vi "Single Tone Audio Measurements.vi"(6 "units settings":T1, 8 "error in":errorcluster, 10 "measurement settings":T4={"Band start"=20.0, "Band stop"=20000.0, "Amplitude"=1.0, "Frequency"=1000.0, "Full scale range"=3.16}, 11 "waveform":waveform(dbl)) -> (0 "error out":errorcluster, 1 "spectrum":cluster{"x0":dbl, "dx":dbl, "magnitude":dbl[]}, 2 "time domain":waveform(dbl), 3 "results":T5)   [LabVIEW 2021]
uses:
  <vilib>/addons/Sound and Vibration/svt_Single Tone Measurements/SoundVib_SingleTone.lvlib
  <vilib>/addons/Sound and Vibration/svt_Distortion/SoundVib_Distortion.lvlib
  controls/single tone audio measurements.ctl
  controls/audio controls.lvlib
  controls/units - ratio.ctl
  <vilib>/addons/Sound and Vibration/svt_Distortion/SVT SNR without Harmonics (Frequency) (1 Ch).vi
  <vilib>/addons/Sound and Vibration/svt_Single Tone Measurements/SVT Dynamic Range (Frequency) (1 Ch).vi
  <vilib>/addons/_NISVFA/_Shared subVIs/Common/SVL Set dB Reference (1 Ch).vi
  <vilib>/addons/Sound and Vibration/svt_Single Tone Measurements/SVT Gain (Time) (1 Ch).vi
  <vilib>/addons/_NISVFA/_Spectrum Processing/SVFA Unit Conversion (Complex) (1 Ch).vi
  <vilib>/addons/Sound and Vibration/svt_Single Tone Measurements/SVT Spurious Free Dynamic Range (Frequency) (1 Ch).vi
  controls/units - snr.ctl
  controls/units settings.ctl
  controls/single tone audio measurement settings.ctl
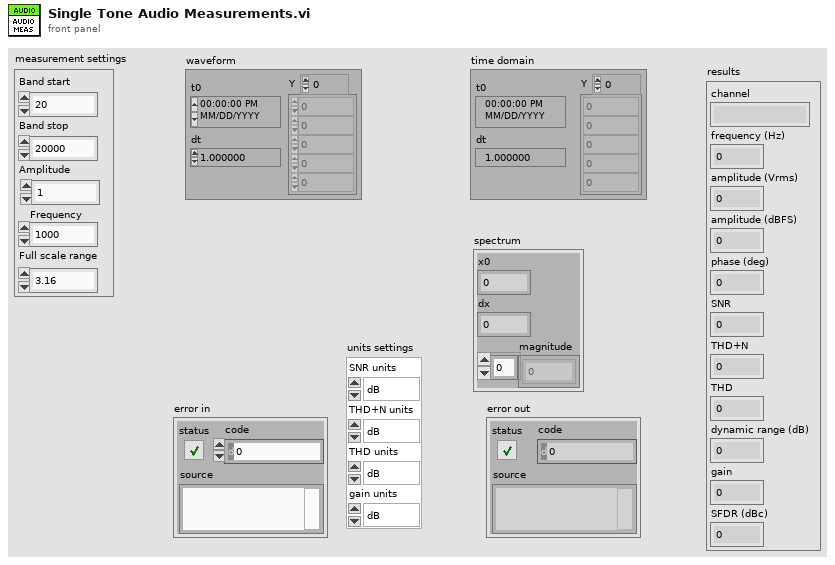
[diagram p1: front panel]
types:
  T1 = typedef "audio controls.lvlib/units settings.ctl" = cluster{"SNR units":T2, "THD+N units":T3, "THD units":T3, "gain units":T3}
  T2 = typedef "audio controls.lvlib/units - snr.ctl" = enum32{"dB", "x/y"}
  T3 = typedef "audio controls.lvlib/units - ratio.ctl" = enum32{"dB", "%", "x/y"}
  T4 = typedef "single tone audio measurement settings.ctl" = cluster{"Band start":dbl, "Band stop":dbl, "Amplitude":dbl, "Frequency":dbl, "Full scale range":dbl}
  T5 = typedef "audio controls.lvlib/single tone audio measurements.ctl" = cluster{"channel":string, "frequency (Hz)":dbl, "amplitude (Vrms)":dbl, "amplitude (dBFS)":dbl, "phase (deg)":dbl, "SNR":dbl, "THD+N":dbl, "THD":dbl, "dynamic range (dB)":dbl, "gain":dbl, "SFDR (dBc)":dbl}
  T6 = enum16{"no change", "spectrum", "spectral density"}
  T7 = cluster{"linear/dB":enum16{"no change", "linear", "dB"}, "dB reference (0: no change)":dbl, "power/magnitude":enum16{"no change", "power", "magnitude"}, "view":enum16{"no change", "rms", "peak", "peak-peak"}}
  T8 = cluster{"start frequency":dbl, "stop frequency":dbl}
  T9 = cluster{"gain units":enum16{"dB", "linear ratio"}, "detected fundamental amplitude units":enum16{"EU rms", "EU peak", "EU peak-peak"}}
  T10 = cluster{"SNR units":enum16{"dB", "linear ratio", "%"}, "detected fundamental amplitude units":enum16{"EU rms", "EU peak", "EU peak-peak"}}
  T11 = typedef "svc_Spectrum Info.ctl" = cluster{"channel name":string, "description":string, "x-axis units":T12, "spectral info":cluster{"spectrum type":T13, "linear/dB":enum16{"linear", "dB"}, "window":u16, "window size":i32, "FFT size":i32}, "engineering units":T14, "custom label":string, "dB reference [EU]":dbl, "peak units":enum16{"rms", "peak", "peak-peak"}, "weighting filter":T15, "spectral density?":bool, "unit label":string, "spectrum skewed?":bool, "complimentary spectrum units":T16}
  T12 = typedef "svc_X-Axis Units.ctl" = u16
  T13 = typedef "svc_Spectrum Type.ctl" = enum16{"FFT Spectrum [complex]", "Amplitude [Magnitude]", "Power [Magnitude^2]", "Cross Spectrum [complex]", "Frequency Response [Complex]"}
  T14 = typedef "svc_Engineering Units Text Ring.ctl" = u16
  T15 = typedef "svc_Weighting Filter Text Ring.ctl" = u16
  T16 = typedef "svc_Complimentary Spectrum Units.ctl" = enum16{"none", "radians", "degrees", "cycles", "imaginary"}
  T17 = cluster{"complex spectrum response":cluster{"f0":dbl, "df":dbl, "complex spectrum":cdb[]}, "spectrum info":T11}
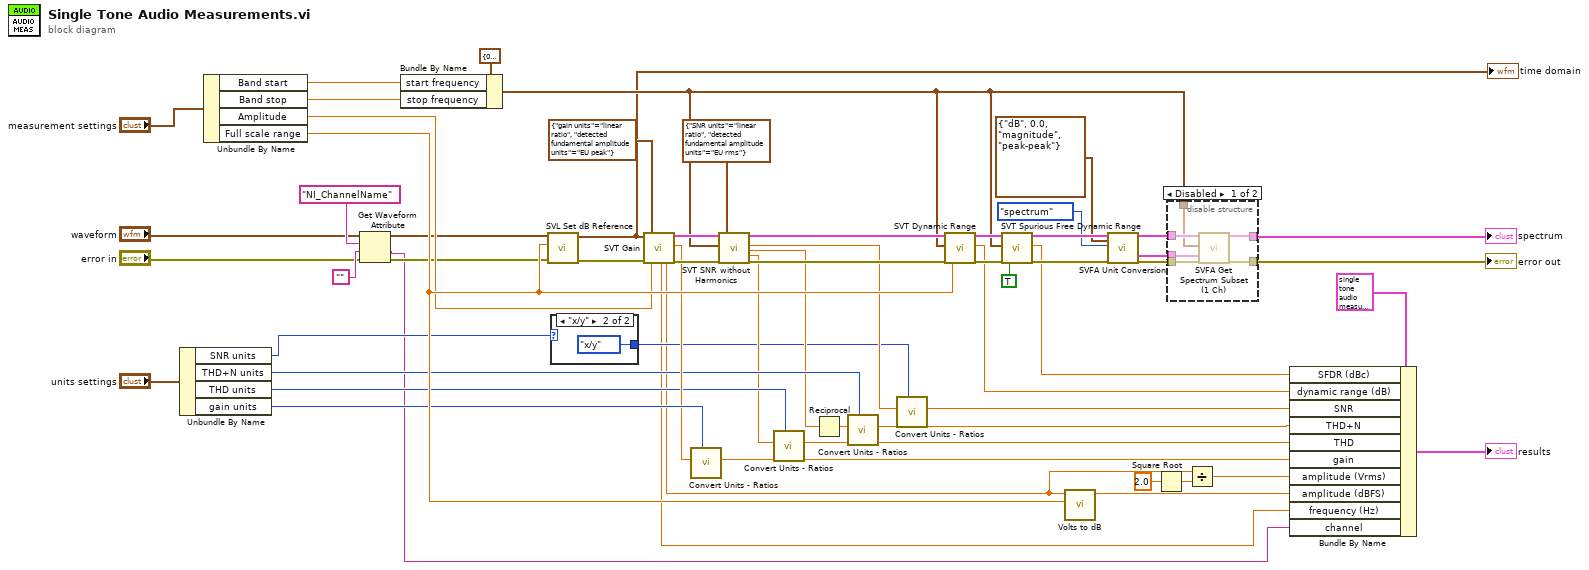
[diagram p0: block diagram]
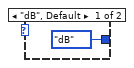
[diagram p2: hidden frame]
diagram:
  n1 = Unbundle By Name("units settings") -> ("SNR units"=w15:T2, "THD+N units"=w24:T3, "THD units"=w18:T3, "gain units"=w27:T3)
  n2 = Unbundle By Name("measurement settings") -> ("Band start"=w58:dbl, "Band stop"=w59:dbl, "Amplitude"=w30:dbl, "Full scale range"=w37:dbl)
  n3 = Get Waveform Attribute(4:"error in", 5:"", 6:"NI_ChannelName" ("name"), 7:"waveform") -> (0:w3:errorcluster, 1:w1:string, 3:w4:waveform(dbl))  [unwired: 1 out]
  n4 = Bundle By Name(cluster=T8 {"start frequency"=0.0, "stop frequency"=0.0} ("frequency range"), "start frequency"=w58, "stop frequency"=w59) -> (w42:T8)
  n5 = call-poly <vilib>:"SVL Set dB Reference.vi"("error in (no error)"=w3, "dB reference [EU]"=w37, "scaled signal in [EU]"=w4) -> ("error out"=w31:errorcluster, "scaled signal out [EU]"=w29:waveform(dbl))  [unwired: 7 in]
  "time domain" <- w29
  n6 = case shown="\"x/y\"" w15 {
    tunnel: [units_-_ratio."dB" ("gain units") units_-_ratio."x/y" ("gain units")] -> w14
    frame "dB", Default {
    }
    frame "x/y" {
    }
  }
  n7 = call-poly <vilib>:"SVT Gain.vi"("scaled signal [EU]"=w29, "error in (no error)"=w31, "desired units"=T9 {"gain units"=enum."linear ratio", "detected fundamental amplitude units"=enum."EU peak"}, "amplitude [EU peak]"=w30) -> ("detected fundamental\nfrequency [Hz]"=w13:dbl, "detected fundamental\namplitude"=w8:dbl, "complex spectrum"=w48:T17, "gain"=w26:dbl, "error out"=w49:errorcluster)  [unwired: 10 in, 1 out]
  n8 = call "Convert Units - Ratios.vi"("gain units"=w27, "linear ratio"=w26) -> ("converted ratio"=w25:dbl)  [unwired: 9 in]
  n9 = call-poly <vilib>:"SVT SNR without Harmonics.vi"("complex spectrum"=w48, "frequency range"=w42, "error in (no error)"=w49, "desired units"=T10 {"SNR units"=enum."linear ratio", "detected fundamental amplitude units"=enum."EU rms"}) -> ("complex spectrum"=w51:T17, "SNR (without harmonics)"=w23:dbl, "SINAD"=w20:dbl, "THD"=w17:dbl, "error out"=w50:errorcluster)  [unwired: 8 in, 3 out]
  n10 = call "Convert Units - Ratios.vi"("gain units"=w18, "linear ratio"=w17) -> ("converted ratio"=w16:dbl)  [unwired: 9 in]
  n11 = Reciprocal(x=w20) -> (1/x=w21:dbl)
  n12 = call "Convert Units - Ratios.vi"("gain units"=w24, "linear ratio"=w21) -> ("converted ratio"=w19:dbl)  [unwired: 9 in]
  n13 = call "Convert Units - Ratios.vi"("gain units"=w14, "linear ratio"=w23) -> ("converted ratio"=w22:dbl)  [unwired: 9 in]
  n14 = call-poly <vilib>:"SVT Dynamic Range.vi"("complex spectrum"=w51, "frequency range"=w42, "error in (no error)"=w50, "full scale amplitude [EU peak]"=w37) -> ("dup complex spectrum"=w54:T17, "dynamic range"=w35:dbl, "error out"=w55:errorcluster)  [unwired: 10 in, 3 out]
  n15 = call-poly <vilib>:"SVT Spurious Free Dynamic Range.vi"("complex spectrum"=w54, "frequency range"=w42, "error in (no error)"=w55, "exclude harmonics"=TRUE) -> ("complex spectrum"=w46:T17, "spurious free dynamic range"=w36:dbl, "error out"=w47:errorcluster)  [unwired: 8 in, 5 out]
  n16 = call "Volts to dB.vi"("Full scale range"=w37, "Voltage(V)"=w8) -> ("Voltage(dB)"=w12:dbl)  [unwired: 9 in]
  n17 = call-poly <vilib>:"SVFA Unit Conversion.vi"("complex spectrum"=w46, "desired scaling"=T7 {"linear/dB"=enum."dB", "dB reference (0: no change)"=0.0, "power/magnitude"=enum."magnitude", "view"=enum."peak-peak"}, "spectral density desired"=T6."spectrum", "error in (no error)"=w47) -> ("converted spectrum"=w43:cluster{"x0":dbl, "dx":dbl, "magnitude":dbl[]}, "spectrum info out"=w40:T11, "error out"=w39:errorcluster)  [unwired: 10 in, 3 out]
  n18 = Square Root(x=2.0 ("y")) -> (sqrt(x)=w11:dbl)
  n19 = disable-structure shown="Disabled" {
    disable-tunnel: w43 -> [w67 w68]
    disable-tunnel: w42 -> [w66 _]
    disable-tunnel: [w65 w69] -> w41
    disable-tunnel: w40 -> [w64 _]
    disable-tunnel: w39 -> [w63 w69]
    disable-tunnel: [w62 w68] -> w32
    frame Disabled {
      n20 = call <vilib>:"SVFA Get Spectrum Subset (1 Ch).vi"("spectrum"=w67, "range"=w66, "spectrum info"=w64, "error in (no error)"=w63) -> ("spectrum subset"=w62:cluster{"x0":dbl, "dx":dbl, "magnitude":dbl[]}, "error out"=w65:errorcluster)  [unwired: 10 in, 4 out]
    }
    frame Enabled {
    }
  }
  "error out" <- w41
  "spectrum" <- w32
  n21 = Divide(x=w8, y=w11) -> (x/y=w9:dbl)
  n22 = Bundle By Name(cluster=T5 {"channel"="", "frequency (Hz)"=0.0, "amplitude (Vrms)"=0.0, "amplitude (dBFS)"=0.0, "phase (deg)"=0.0, "SNR"=0.0, "THD+N"=0.0, "THD"=0.0, "dynamic range (dB)"=0.0, "gain"=0.0, "SFDR (dBc)"=0.0} ("results"), "SFDR (dBc)"=w36, "dynamic range (dB)"=w35, "SNR"=w22, "THD+N"=w19, "THD"=w16, "gain"=w25, "amplitude (Vrms)"=w9, "amplitude (dBFS)"=w12, "frequency (Hz)"=w13, "channel"=w1) -> (→"results":T5)
